vi "Write.vi"(8 "error in (no error)":errorcluster, 9 "timeout (ms)":i32=1000, 10 "pcap CAN DATA in":u8[](array[numeric]), 11 "XNET_CAN_RW in":refnum<class "XNET CAN RW.lvclass">) -> (0 "error out":errorcluster, 3 "XNET_CAN_RW out":refnum<class "XNET CAN RW.lvclass">, 4 "number written":i32=-1)   [LabVIEW 2021, in "XNET CAN RW.lvclass"]
uses:
  XNET CAN RW.lvclass
  XNET CAN RW.lvclass/XNET CAN RW.ctl
  <vilib>/xnet/xnet.llb/XNET Write (Frame CAN).vi
  <vilib>/CIF Foundation/CIF CAN RW Core/CAN_RW_CORE.lvclass
  C:/Program Files/National Instruments/LabVIEW 2021/vi.lib/CIF Foundation/CIF CAN RW Core/CAN_RW_CORE.lvclass
  D:/dev/Packages/CAN_RW_XNET/src/XNET CAN RW.lvclass
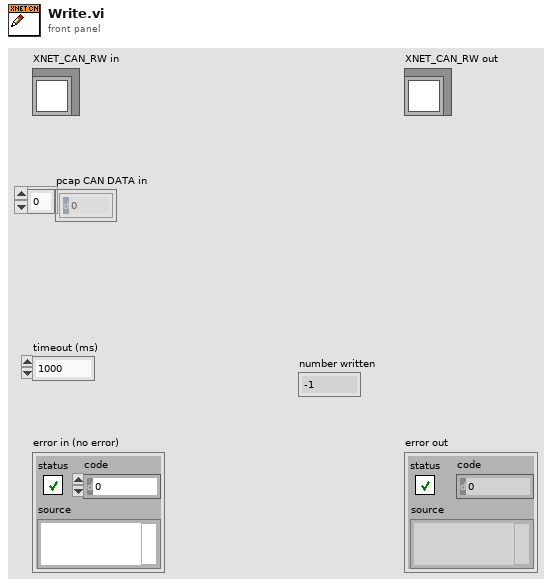
[diagram p1: front panel]
types:
  T1 = typedef "XNET Frame CAN.ctl" = cluster{"timestamp":timestamp, "payload":u8[], "identifier":u32, "type":T2, "extended?":bool, "echo?":bool}
  T2 = typedef "XNET Frame Type CAN.ctl" = u8
  T3 = typedef "CAN_RW_CORE.lvclass/CAN Port Configuration.ctl" = cluster{"Mode":T4, "Baud Rate":u64, "Temination On":bool, "Subordinate":bool, "Echo TX":bool, "FD Config":T5}
  T4 = typedef "CAN_RW_CORE.lvclass/CAN Mode.ctl" = enum16{"CAN 2.0", "CAN FD"}
  T5 = typedef "CAN_RW_CORE.lvclass/FD Config.ctl" = cluster{"FD Baud Rate":u64, "ISO Mode":bool, "BRS Enabled":bool}
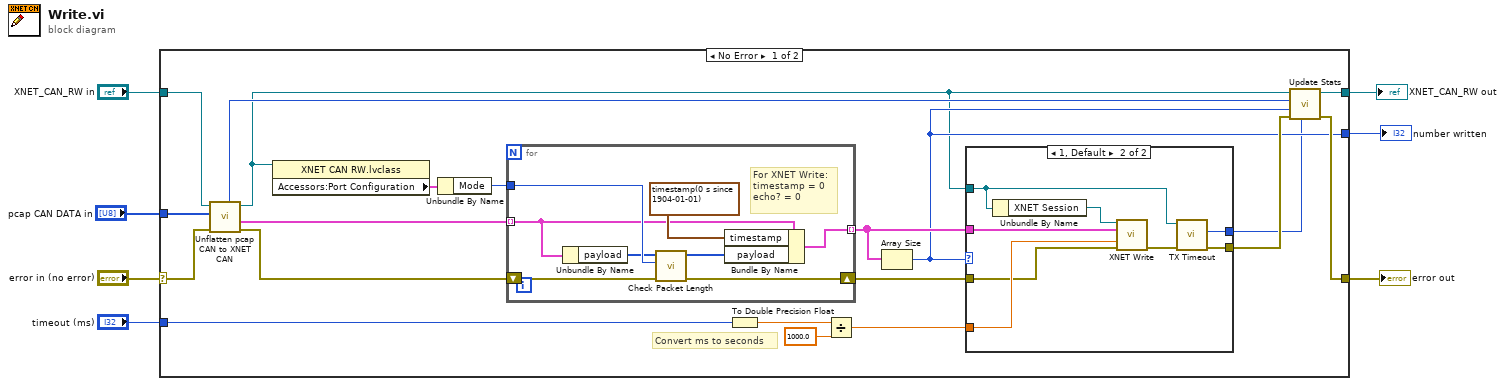
[diagram p0: block diagram]
diagram:
  n1 = case shown="No Error" "error in (no error)" {
    selector: "error in (no error)" -> [w17 w46]
    tunnel: [w12 w46] -> w6
    tunnel: [w14 w45] -> w4
    tunnel: "XNET_CAN_RW in" -> [w15 w45]
    tunnel: "pcap CAN DATA in" -> [w19 _]
    tunnel: "timeout (ms)" -> [w24 _]
    tunnel: [w10 _] -> w1
    frame No Error {
      # "Convert ms to seconds"
      n2 = call "Unflatten pcap CAN to XNET CAN.vi"("error in (no error)"=w17, "pcap CAN DATA in"=w19, "XNET_CAN_RW in"=w15) -> ("error out"=w16:errorcluster, "XNET CAN Data"=w18:T1[], "XNET_CAN_RW out"=w9:refnum<class "XNET CAN RW.lvclass">, "Number Filtered"=w11:u32)  [unwired: 3 in, 2 out]
      n3 = property class="XNET CAN RW.lvclass"(reference=w9) -> ("Accessors:Port Configuration"=w20:T3)  [unwired: 1 in, 2 out]
      n4 = Unbundle By Name(w20) -> ("Mode"=w21:T4)
      n5 = for {
        tunnel: [w44] -> w27 mode=indexing
        shift-right: [w41] -> w22
        shift-left: w16 -> [w42]
        tunnel: w21 -> [w40]
        tunnel: w18 -> [w37] mode=indexing
        # "For XNET Write:\ntimestamp = 0\necho? = 0"
        n6 = Unbundle By Name(w37) -> ("payload"=w39:u8[])
        n7 = call "Check Packet Length.vi"("error in (no error)"=w42, "Mode"=w40, "payload in"=w39) -> ("error out"=w41:errorcluster, "payload out"=w43:u8[])  [unwired: 7 in]
        n8 = Bundle By Name(cluster=w37, "timestamp"=timestamp(0 s since 1904-01-01), "payload"=w43) -> (w44:T1)
      }
      n9 = To Double Precision Float(number=w24) -> (double precision float=w26:dbl)
      n10 = Divide(x=w26, y=1000.0) -> (x/y=w23:dbl)
      n11 = Array Size(array=w27) -> (size(s)=w10:i32)
      n12 = case shown="1, Default" w10 {
        tunnel: w22 -> [w28 w32]
        tunnel: [w28 w33] -> w13
        tunnel: w27 -> [_ w36]
        tunnel: w23 -> [_ w35]
        tunnel: w9 -> [_ w31]
        tunnel: [_ w29] -> w8
        frame 0 {
        }
        frame 1, Default {
          n13 = Unbundle By Name(w31) -> ("XNET Session"=w30:refnum<k21>)
          n14 = call-poly <vilib>:"XNET Write.vi"("session in"=w30, "data"=w36, "timeout (10)"=w35, "error in (no error)"=w32) -> ("error out"=w34:errorcluster)  [unwired: 10 in, 1 out]
          n15 = call "TX Timeout.vi"("error in (no error)"=w34, "XNET_CAN_RW in"=w31) -> ("error out"=w33:errorcluster, "ACK Errors"=w29:u32)  [unwired: 8 in]
        }
      }
      n16 = call <vilib>:"Update Stats.vi"("ACK Errors"=w8, "error in (no error)"=w13, "Number Read"=w10, "Number Filtered"=w11, "CAN_RW_CORE in"=w9) -> ("error out"=w12:errorcluster, "CAN_RW_CORE out"=w14:refnum<class "XNET CAN RW.lvclass">)  [unwired: 5 in]
    }
    frame Error {
    }
  }
  "error out" <- w6
  "XNET_CAN_RW out" <- w4
  "number written" <- w1
